vi "Wifi_USRP_Tx_chat_deneme.vi"() -> ()   [LabVIEW 2024]
uses:
  <vilib>/Analysis/2dsp.llb/Inverse Complex FFT.vi
  <vilib>/addons/Modulation/Digital/Channel Coding/MT Convolutional Encoder (Rate).vi
  <vilib>/addons/Modulation/Digital/Support/Common/Validators/mod_Generate Bits Validate.vi
  <vilib>/addons/Modulation/Digital/General/subVIs/mod_Generate Bits Pattern.vi
  <vilib>/addons/Modulation/Analog/support/mod_Set Error Source.vi
  <vilib>/addons/Modulation/Digital/Support/Common/Validators/mod_Validate Bit Stream.vi
  <vilib>/addons/Modulation/Digital/Channel Coding/Convolutional codes/mod_Convolutional encoder.vi
  <vilib>/addons/Modulation/Digital/Support/Common/Validators/mod_Validate Number of Rows Columns.vi
  <vilib>/addons/Modulation/Digital/Channel Coding/Block codes/subVIs/mod_Buffer block code info.vi
  <vilib>/addons/Modulation/Digital/Interleaving/Block Interleaver/mod_Block Interleaver (Matrix).vi
  <vilib>/addons/Modulation/Digital/Channel Coding/Convolutional codes/subVIs/mod_Generate encoder tap connections.vi
  <vilib>/addons/Modulation/Digital/Channel Coding/Convolutional codes/subVIs/mod_Perform convolutional encoding.vi
  <vilib>/addons/Modulation/Digital/Channel Coding/Block codes/subVIs/mod_Buffer block code info (I8).vi
  <vilib>/addons/Modulation/Digital/Channel Coding/Convolutional codes/subVIs/mod_Generate valid reset (convolutional, I8).vi
  <vilib>/addons/Modulation/Digital/General/subVIs/mod_Generate Bits PN Sequence.vi
  <vilib>/addons/Modulation/Digital/Channel Coding/Convolutional codes/subVIs/mod_Select known generator matrix.vi
  <vilib>/addons/Modulation/Digital/Support/Common/Validators/mod_Validate Convolutional Encoder prms.vi
  <vilib>/addons/Modulation/Digital/General/MT Map Bits to QAM Symbols.vi
  <vilib>/addons/Modulation/Digital/General/MT Map Bits to PSK Symbols.vi
  <instrlib>/niUSRP/niUSRP Write Tx Data (CDB).vi
  <vilib>/Analysis/NI_AALPro.lvlib
  <vilib>/addons/Modulation/niDMT.lvlib
panel:
  out "Waveform Graph":dbl[](graph)
  in  "stop":bool
  out "?":string="Please write a message"
  in  "Send":bool
  out "appended array":cdb[](array[numeric])
  out "FFT(x)":dbl[](graph)
  out "Phase":dbl[](graph)
  out "message bitstream":i8[](array[numeric])
  out "Header and payload symbols concetanated":cdb[][](array[numeric])
  out "Pilot polarities":dbl[][](array[numeric])
  out "Header symbols":cdb[](array[numeric]) format="%.3f"
  out "0, 1":i16
  in  "bit order":enum16{"MSB first", "LSB first"}(ring)=enum."LSB first"
  out "Message Length (bits)":i32
  in  "text message":string
  out "LLTF":cdb[](array[numeric])
  out "LSTF":cdb[](array[numeric])
  in  "Tab Control":enum32{"Parameters", "Debug"}(tab)
  in  "device names":refnum<k15>="192.168.10.2"
  in  "IQ rate":dbl=5000000.0 format="%#_6p"
  in  "gain":dbl=9.0 format="%#_6f"
  in  "carrier frequency":dbl=910000000.0 format="%#_6p"
  out "coerced IQ rate":dbl=100000.0 format="%#_6p"
  in  "active antenna":string="TX1"
  in  "error in (no error)":errorcluster
  out "error out":errorcluster
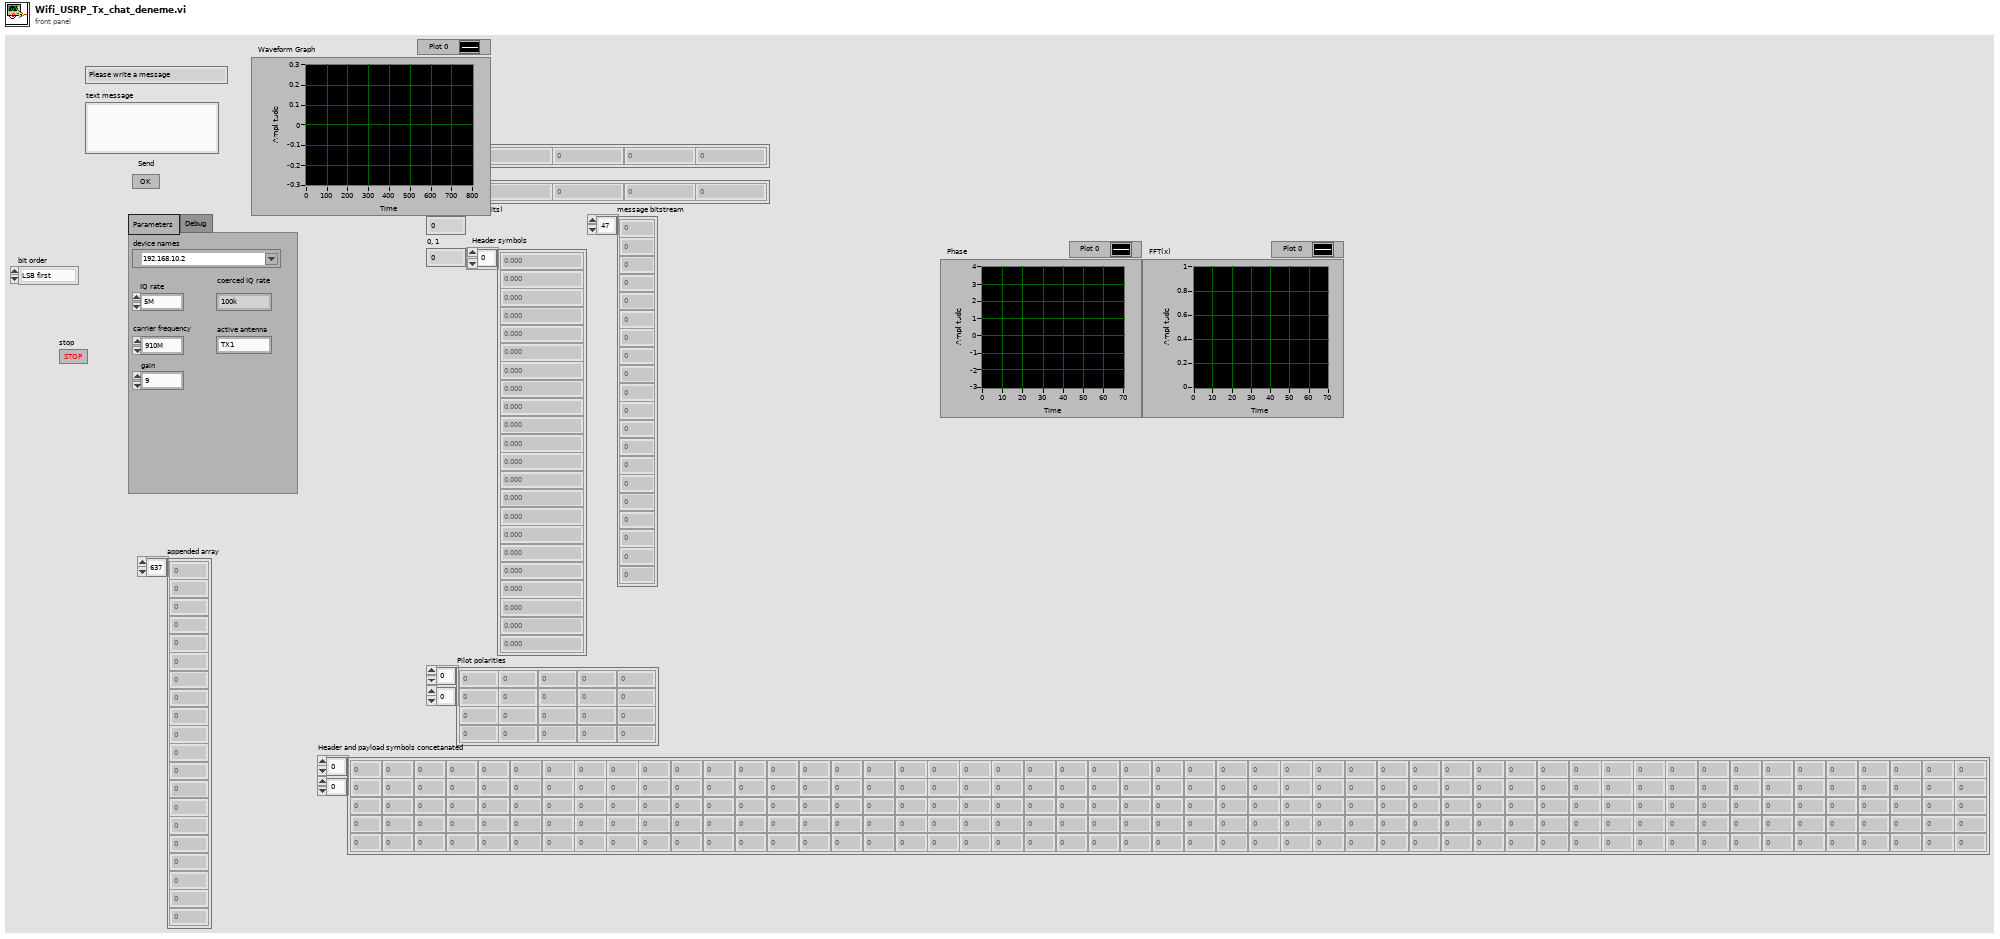
[diagram p1: front panel]
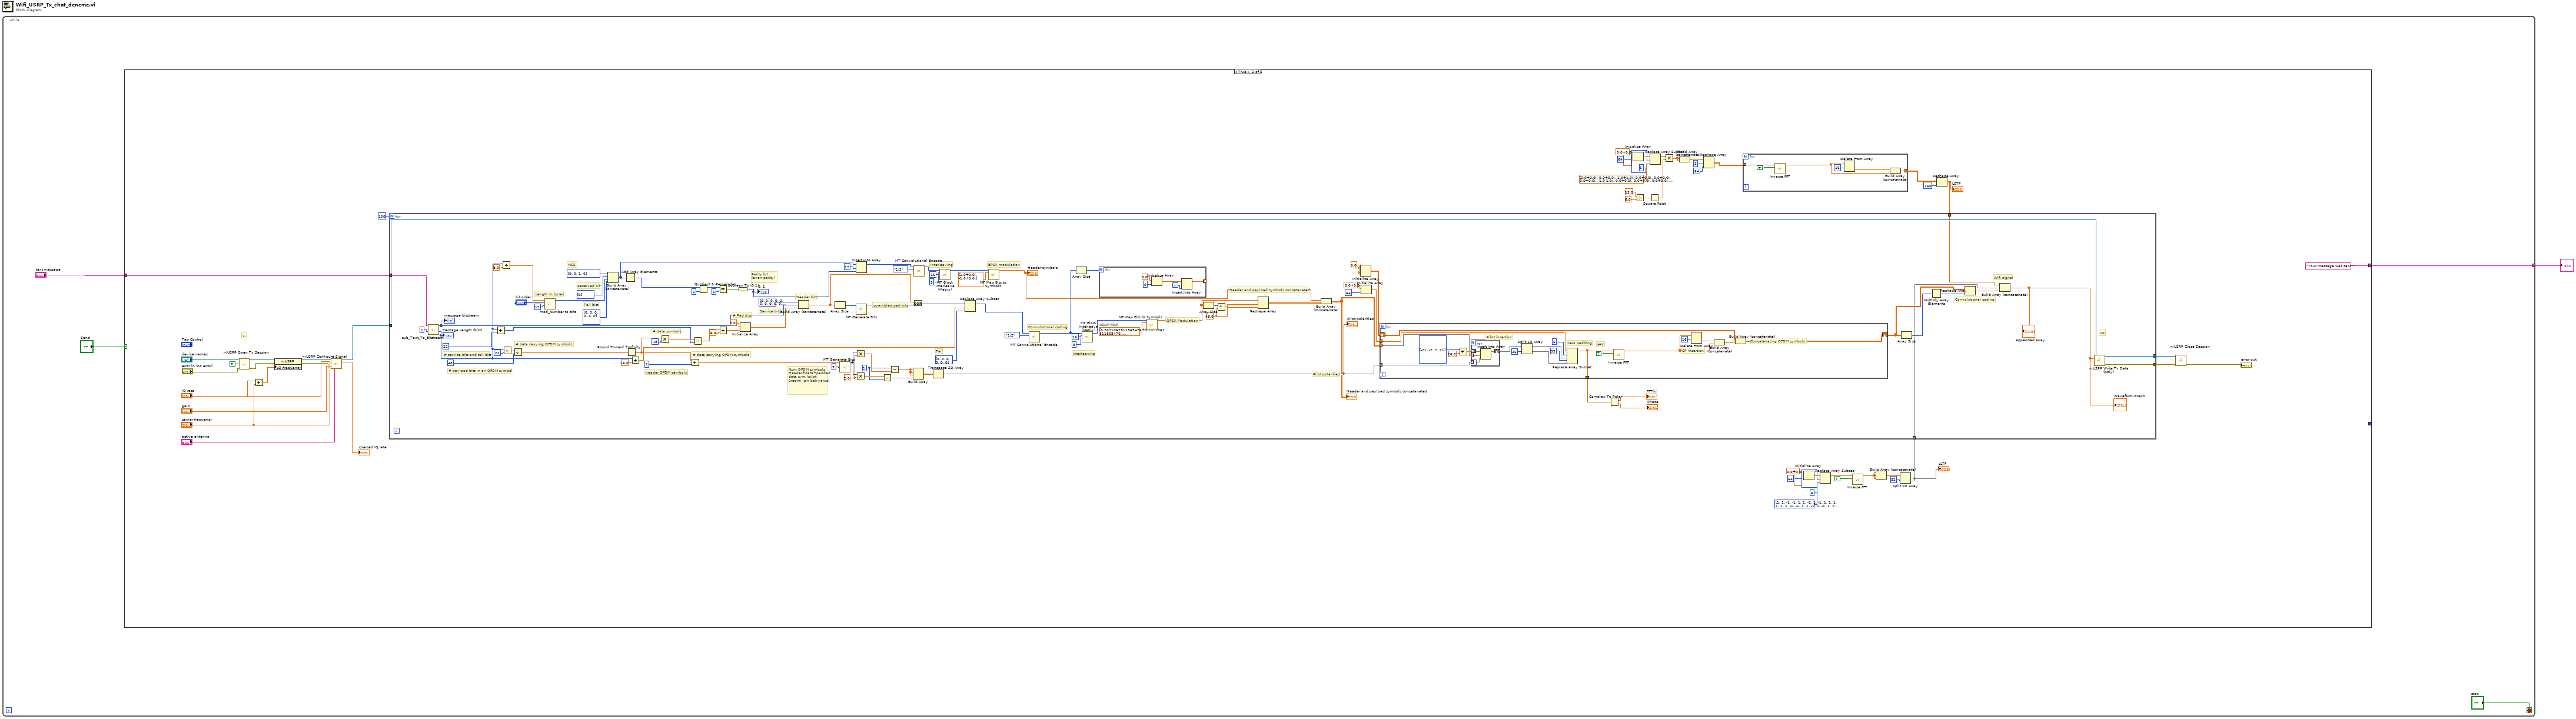
[diagram p0: block diagram]
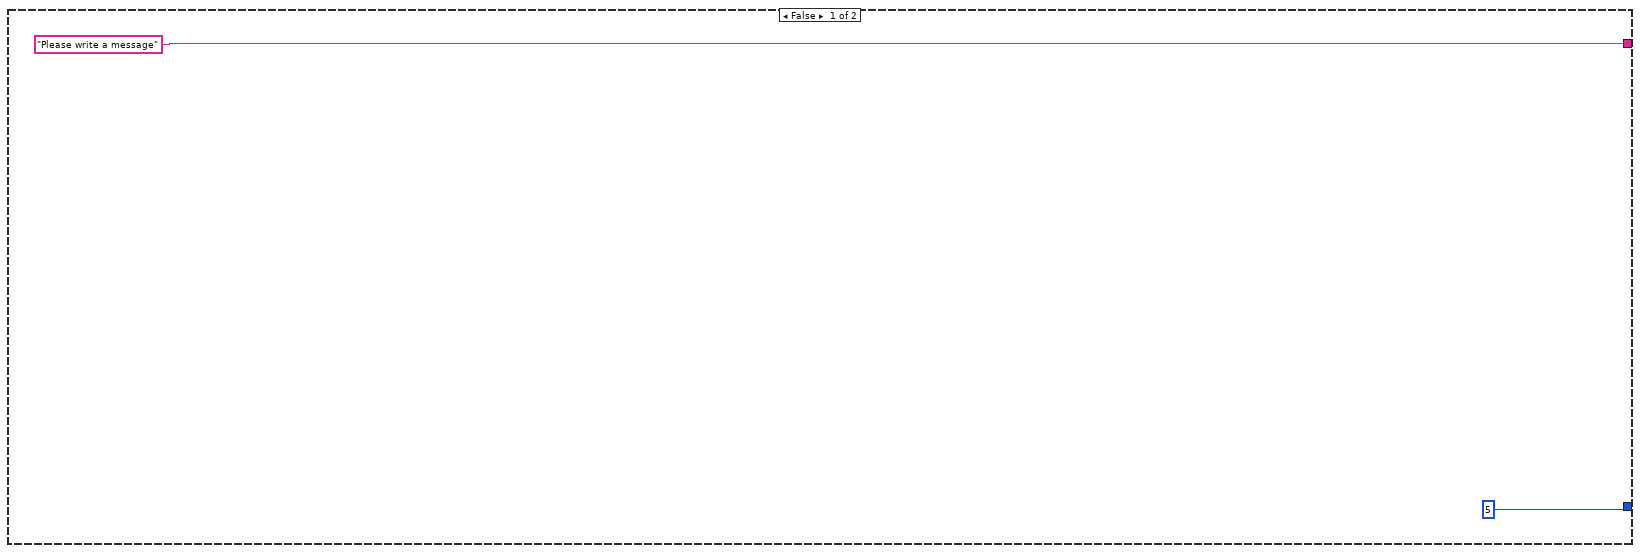
[diagram p2: hidden frame]
diagram:
  n1 = while {
    tunnel: [w2] -> w1
    stop <- "stop" stop-if-true
    n2 = case shown="True" "Send" {
      tunnel: ["Please write a message" "Your message was sent."] -> w2
      tunnel: "text message" -> [_ w9]
      tunnel: [5 _] -> _
      frame False {
      }
      frame True {
        # "1."
        n3 = call <instrlib>:"niUSRP Open Tx Session.vi"("device names"="device names", "reset"=TRUE, "error in (no error)"="error in (no error)") -> ("session handle out"=w45:refnum<k15>, "error out"=w46:errorcluster)  [unwired: 11 in]
        n4 = Add(x="IQ rate", y="carrier frequency") -> (x+y=w40:dbl)
        n5 = property class="niUSRP"(reference=w45, error in=w46, "LO Frequency"=w40) -> (reference out=w48:refnum<k15>, error out=w47:errorcluster)
        n6 = call <instrlib>:"niUSRP Configure Signal.vi"("session handle"=w48, "IQ rate"="IQ rate", "carrier frequency"="carrier frequency", "gain"="gain", "error in (no error)"=w47, "active antenna"="active antenna") -> ("session handle out"=w44:refnum<k15>, "coerced IQ rate"=→"coerced IQ rate":dbl)  [unwired: 5 in, 3 out]
        n7 = Initialize Array(cdb 0.0+0.0i ("element"), 64 ("dimension size")) -> (w32:cdb[])
        n8 = Divide(x=13.0, y=6.0) -> (x/y=w36:dbl)
        n9 = Square Root(x=w36) -> (sqrt(x)=w37:dbl)
        n10 = Replace Array Subset(array=w32, new element=cdb[] [0.0+0.0i, 0.0+0.0i, 1.0+1.0i, 0.0+0.0i, 0.0+0.0i, 0.0+0.0i, -1.0-1.0i, 0.0+0.0i, 0.0+0.0i, 0.0+0.0i, 1.0+1.0i, 0.0+0.0i, 0.0+0.0i, 0.0+0.0i, -1.0-1.0i, 0.0+0.0i, 0.0+0.0i, 0.0+0.0i, -1.0-1.0i, 0.0+0.0i, 0.0+0.0i, 0.0+0.0i, 1.0+1.0i, 0.0+0.0i, 0.0+0.0i, 0.0+0.0i, 0.0+0.0i, 0.0+0.0i, 0.0+0.0i, 0.0+0.0i, -1.0-1.0i, 0.0+0.0i, 0.0+0.0i, 0.0+0.0i, -1.0-1.0i, 0.0+0.0i, 0.0+0.0i, 0.0+0.0i, 1.0+1.0i, 0.0+0.0i, 0.0+0.0i, 0.0+0.0i, 1.0+1.0i, 0.0+0.0i, 0.0+0.0i, 0.0+0.0i, 1.0+1.0i, 0.0+0.0i, 0.0+0.0i, 0.0+0.0i, 1.0+1.0i, 0.0+0.0i, 0.0+0.0i], index=6) -> (w38:cdb[])
        n11 = Multiply(x=w38, y=w37) -> (x*y=w39:cdb[])
        n12 = Build Array (concatenate)(w39, w39) -> (w33:cdb[])
        n13 = Reshape Array(w33, 2 ("dimension size"), 64 ("dimension size")) -> (w34:cdb[][])
        n14 = for {
          tunnel: w34 -> [w185] mode=indexing
          tunnel: [w181] -> w35 mode=indexing
          n15 = call-poly <vilib>:"Inverse FFT.vi"("shift?"=TRUE, "FFT {X}"=w185) -> ("X"=w182:cdb[])  [unwired: 8 in, 1 out]
          n16 = Delete From Array(array=w182, length=16) -> (deleted portion=w183:cdb[])  [unwired: 1 in, 1 out]
          n17 = Build Array (concatenate)(w183, w182) -> (w181:cdb[])
        }
        n18 = Initialize Array(cdb 0.0+0.0i ("element"), 64 ("dimension size")) -> (w18:cdb[])
        n19 = Replace Array Subset(array=w18, new element=i32[] [1, 1, -1, -1, 1, 1, -1, 1, -1, 1, 1, 1, 1, 1, 1, -1, -1, 1, 1, -1, 1, -1, 1, 1, 1, 1, 0, 1, -1, -1, 1, 1, -1, 1, -1, 1, -1, -1, -1, -1, -1, 1, 1, -1, -1, 1, -1, 1, -1, 1, 1, 1, 1], index=6) -> (w21:cdb[])
        n20 = call-poly <vilib>:"Inverse FFT.vi"("shift?"=TRUE ("shift? 3"), "FFT {X}"=w21) -> ("X"=w19:cdb[])  [unwired: 8 in, 1 out]
        n21 = Build Array (concatenate)(w19, w19, w19) -> (w20:cdb[])
        n22 = Split 1D Array(array=w20, index=32) -> (second subarray=w11:cdb[])  [unwired: 1 out]
        "LLTF" <- w11
        n23 = Reshape Array(w35, 160 ("dimension size")) -> (w22:cdb[])
        "LSTF" <- w22
        n24 = for {
          N: 100 -> [_]
          tunnel: w44 -> [w150]
          tunnel: [w149] -> w55
          tunnel: [w148] -> w54
          tunnel: w9 -> [w63]
          tunnel: w22 -> [w62]
          tunnel: w11 -> [w61]
          w66 = 48.0 ("y")
          w111 = cdb[] [0.7071067811865476+0.7071067811865476i, 0.7071067811865476-0.7071067811865476i, -0.7071067811865476+0.7071067811865476i, -0.7071067811865476-0.7071067811865476i]  # 4QAM MAP
          w140 = 0.0 ("element")
          w135 = 2.0 ("y")
          w134 = 1
          # "# data carrying OFDM symbols"
          # "Service bits"
          # "# Pad bits"
          # "# service bits and tail bits"
          # "# data symbols"
          # "# data carrying OFDM symbols"
          # "# payload bits in an OFDM symbol"
          # "Interleaving"
          # "Pilot polarities"
          # "header OFDM sembolü"
          # "Wifi signal"
          # "Convolutional coding"
          # "Interleaving"
          # "scrambled pad bits"
          # "Tail"
          # "QPSK Modulation"
          # "BPSK modulation"
          # "Convolutional coding"
          # "Header and payload symbols concetanated"
          # "Header bits"
          # "Parity bit (even parity)"
          # "Tail bits"
          # "Length in bytes"
          # "Reserved bit"
          # "MCS"
          # "Num OFDM symbols\nHeader+data+padded data sym (pilot üretimi için bakıyoruz)"
          # "10."
          n25 = call "sub_Text_To_Bitstream.vi"("Packet\nMessage Length (bits)"=1 ("Packet\nMessage Length (bits)"), "text"=w63) -> ("File Length (bits)"=w80:i32, "message bitstream"=w87:i8[])  [unwired: 7 in, 1 out]
          "Message Length (bits)" <- w80
          "message bitstream" <- w87
          n26 = Add(x=w80, y=22) -> (x+y=w92:i32)
          n27 = Divide(x=w80, y=8.0) -> (x/y=w131:dbl)
          n28 = Add(x=w80, y=22) -> (x+y=w90:i32)
          n29 = Divide(x=w90, y=48) -> (x/y=w88:dbl)
          n30 = call <vilib>:"mod_Number to Bits.vi"("number of bits"=12, "bit order"="bit order", "Number"=w131) -> ("bits"=w126:i8[])  [unwired: 8 in]
          n31 = Build Array (concatenate)(i32[] [0, 0, 1, 0], i32[] [0], w126, i32[] [0, 0, 0, 0, 0, 0]) -> (w120:i32[])
          n32 = Add Array Elements(numeric array=w120) -> (sum=w118:i32)
          n33 = Round Toward +Infinity(x=w88) -> (ceil(x): smallest int >= x=w72:dbl)
          n34 = Add(x=w80, y=16.0) -> (x+y=w74:dbl)
          n35 = Multiply(x=w72, y=48) -> (x*y=w94:dbl)
          n36 = Add(x=w72, y=1 ("value")) -> (x+y=w70:dbl)
          n37 = Subtract(x=w94, y=w92) -> (x-y=w79:dbl)
          n38 = Quotient & Remainder(x=w118, y=2) -> (x-y*floor(x/y)=w123:i32)  [unwired: 1 out]
          n39 = Equal?(x=w123, y=1) -> (x = y?=w121:bool)
          n40 = Add(x=w79, y=6.0) -> (x+y=w77:dbl)
          n41 = Boolean To (0,1)(Boolean=w121) -> (0, 1=w117:i16)
          "0, 1" <- w117
          n42 = Initialize Array(0.0 ("element"), w77) -> (w84:dbl[])
          n43 = Build Array (concatenate)(i32[] [0, 0, 0, 0, 0, 0, 0, 0, 0, 0, 0, 0, 0, 0, 0, 0], w87, w84) -> (w73:dbl[])
          n44 = Array Size(array=w73) -> (size(s)=w83:i32)
          n45 = call <vilib>:"MT Generate Bits.vi"("total bits (128)"=w70, "PN sequence order (9)"=9) -> ("output bit stream"=w145:i8[])  [unwired: 11 in, 2 out]
          n46 = Multiply(x=w145, y=w135) -> (x*y=w146:dbl[])
          n47 = Multiply(x=w145, y=w135) -> (x*y=w144:dbl[])
          n48 = Insert Into Array(array=w120, index=17, new element=w117) -> (w115:i32[])
          n49 = call <vilib>:"MT Generate Bits.vi"("total bits (128)"=w83) -> ("output bit stream"=w82:i8[])  [unwired: 12 in, 2 out]
          n50 = Subtract(x=w144, y=w134) -> (x-y=w142:dbl[])
          n51 = Subtract(x=w134, y=w146) -> (x-y=w143:dbl[])
          n52 = Exclusive Or(1:w82, 2:w73) -> (0:w76:i32[])
          n53 = Build Array(w143, w143, w143, w142) -> (w141:dbl[][])
          n54 = call-poly <vilib>:"MT Convolutional Encode.vi"("input bit stream"=w115, "rate (k/n)"=enum16{"1/2", "1/3", "1/4", "2/3", "3/4"}."1/2") -> ("output bit stream"=w97:i8[])  [unwired: 11 in, 2 out]
          n55 = Transpose 2D Array(2D array=w141) -> (transposed array=w101:dbl[][])
          "Pilot polarities" <- w101
          n56 = call <vilib>:"MT Block Interleave (Matrix).vi"("data in"=w97, "number of rows"=16, "number of columns"=3) -> ("data out"=w96:i32[])  [unwired: 11 in, 1 out]
          n57 = Replace Array Subset(array=w76, new element=i32[] [0, 0, 0, 0, 0, 0], index=w74) -> (w69:i32[])
          n58 = call-poly <vilib>:"MT Map Bits to Symbols.vi"("input bit stream"=w96, "symbol map"=cdb[] [1.0+0.0i, -1.0+0.0i]) -> ("symbols"=w106:cdb[])  [unwired: 12 in, 1 out]
          "Header symbols" <- w106
          n59 = call-poly <vilib>:"MT Convolutional Encode.vi"("input bit stream"=w69, "rate (k/n)"=enum16{"1/2", "1/3", "1/4", "2/3", "3/4"}."1/2") -> ("output bit stream"=w68:i8[])  [unwired: 11 in, 2 out]
          n60 = Array Size(array=w68) -> (size(s)=w103:i32)
          n61 = call <vilib>:"MT Block Interleave (Matrix).vi"("data in"=w68, "number of rows"=16, "number of columns"=3) -> ("data out"=w102:i32[])  [unwired: 11 in, 1 out]
          n62 = for {
            N: w103 -> [_]
            tunnel: [w151] -> _ mode=indexing
            i -> [w155]
            n63 = Initialize Array(0.0 ("element"), 0 ("dimension size")) -> (w154:dbl[])
            n64 = Insert Into Array(array=w154, new element=w155) -> (w151:dbl[])  [unwired: 1 in]
          }
          n65 = call-poly <vilib>:"MT Map Bits to Symbols.vi"("input bit stream"=w102, "symbol map"=w111) -> ("symbols"=w110:cdb[])  [unwired: 12 in, 1 out]
          n66 = Array Size(array=w110) -> (size(s)=w109:i32)
          n67 = Divide(x=w109, y=w66) -> (x/y=w65:dbl)
          n68 = Reshape Array(w110, w65, w66) -> (w64:cdb[][])
          n69 = Build Array (concatenate)(w106, w64) -> (w67:cdb[][])
          "Header and payload symbols concetanated" <- w67
          n70 = Initialize Array(w140, w140, w140) -> (w139:dbl[][])
          n71 = Initialize Array(cdb 0.0+0.0i ("element"), 64 ("dimension size")) -> (w136:cdb[])
          n72 = for {
            tunnel: w67 -> [w172] mode=indexing
            tunnel: w101 -> [w171] mode=indexing
            shift-right: [w169] -> w105
            shift-left: w139 -> [w170]
            tunnel: w136 -> [w162]
            tunnel: [w156] -> w58
            # "Concatenating OFDM symbols"
            # "CP insertion"
            # "IFFT"
            # "Zero padding"
            # "Pilot insertion"
            n73 = Add(x=i32[] [-21, -7, 7, 21], y=26.0) -> (x+y=w173:dbl[])
            n74 = for {
              tunnel: w173 -> [w179] mode=indexing
              shift-right: [w177] -> w167
              shift-left: w172 -> [w178]
              tunnel: w171 -> [w176] mode=indexing
              n75 = Insert Into Array(array=w178, index=w179, new element=w176) -> (w177:cdb[])
            }
            n76 = Split 1D Array(array=w167, index=26) -> (first subarray=w165:cdb[], second subarray=w164:cdb[])
            n77 = Replace Array Subset(array=w162, new element #1=w165, index #1=6 ("index"), new element #2=w164, index #2=33 ("index")) -> (w156:cdb[])
            n78 = call-poly <vilib>:"Inverse FFT.vi"("shift?"=TRUE, "FFT {X}"=w156) -> ("X"=w157:cdb[])  [unwired: 8 in, 1 out]
            n79 = Delete From Array(array=w157, length=16) -> (deleted portion=w158:cdb[])  [unwired: 1 in, 1 out]
            n80 = Build Array (concatenate)(w158, w157) -> (w159:cdb[])
            n81 = Build Array (concatenate)(w170, w159) -> (w169:cdb[][])
          }
          n82 = Complex To Polar(r * e^(i*theta)=w58) -> (r=→"FFT(x)":dbl[], theta=→"Phase":dbl[])
          n83 = Array Size(array=w105) -> (size(s)=w104:i32[])
          n84 = Multiply Array Elements(1:w104) -> (0:w113:i32)
          n85 = Reshape Array(w105, w113) -> (w100:cdb[])
          n86 = Build Array (concatenate)(w62, w61, w100) -> (w57:cdb[])
          "appended array" <- w57
          "Waveform Graph" <- w57
          n87 = call-poly <instrlib>:"niUSRP Write Tx Data (poly).vi"("session handle"=w150, "data"=w57) -> ("session handle out"=w148:refnum<k15>, "error out"=w149:errorcluster)  [unwired: 12 in]
        }
        n88 = call <instrlib>:"niUSRP Close Session.vi"("session handle"=w54, "error in (no error)"=w55) -> ("error out"=→"error out":errorcluster)  [unwired: 13 in]
      }
    }
  }
  "?" <- w1
